vi "Switch Scalar Type.vi"(8 "error in (no error)":errorcluster, 11 "Node Ptr":u64 format="%.0x") -> (0 "error out":errorcluster)   [LabVIEW 2019, in "FPGA Addon System Explorer.lvlib"]
uses:
  FPGA Addon System Explorer.lvlib
  <vilib>/NI VeriStand/Custom Device API/Custom Device Channel.ctl
  <vilib>/NI VeriStand/Custom Device API/Custom Device Channel Type.ctl
  Addon Shared/SubVIs/Constants.vi
  <vilib>/NI VeriStand/Custom Device API/Set Item Property (String).vi
  <vilib>/NI VeriStand/Custom Device API/Get Item Property (String).vi
  <vilib>/NI VeriStand/Custom Device API/Custom Device API.lvlib
  Addon Shared/FPGA Addon Shared.lvlib
  <vilib>/NI VeriStand/Custom Device Tools/Custom Device Utility Library/Custom Device Utility Library.lvlib
  <vilib>/NI VeriStand/Custom Device Tools/Custom Device Utility Library/Search Direction.ctl
  <vilib>/NI VeriStand/Custom Device Tools/Custom Device Utility Library/NI VeriStand - Search for Item by GUID.vi
panel:
  in  "Tag":string
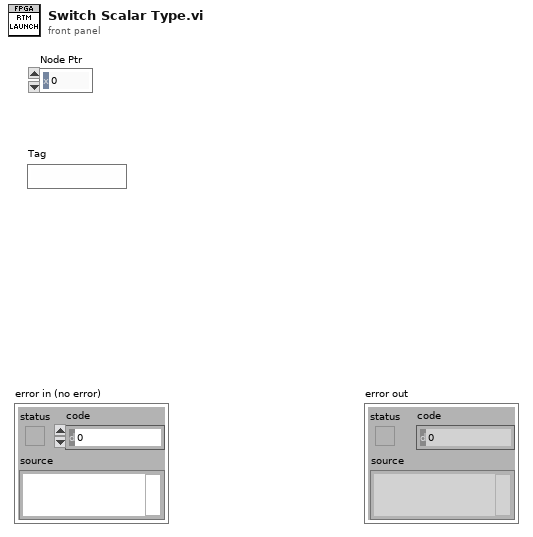
[diagram p1: front panel]
types:
  T1 = typedef "Custom Device Utility Library.lvlib/Search Direction.ctl" = enum16{"Down", "Up"}
  T2 = typedef "Custom Device API.lvlib/Custom Device Item Ref.ctl" = u64
  T3 = typedef "Custom Device API.lvlib/Custom Device Item Info.ctl" = cluster{"Name":string, "Is Channel":bool, "GUID":string, "Is Waveform":bool}
  T4 = typedef "Custom Device API.lvlib/Custom Device Channel.ctl" = cluster{"Type":T5, "Units":string, "Default Value":dbl, "Faultable":bool, "Scalable":bool}
  T5 = typedef "Custom Device API.lvlib/Custom Device Channel Type.ctl" = enum16{"Input", "Output"}
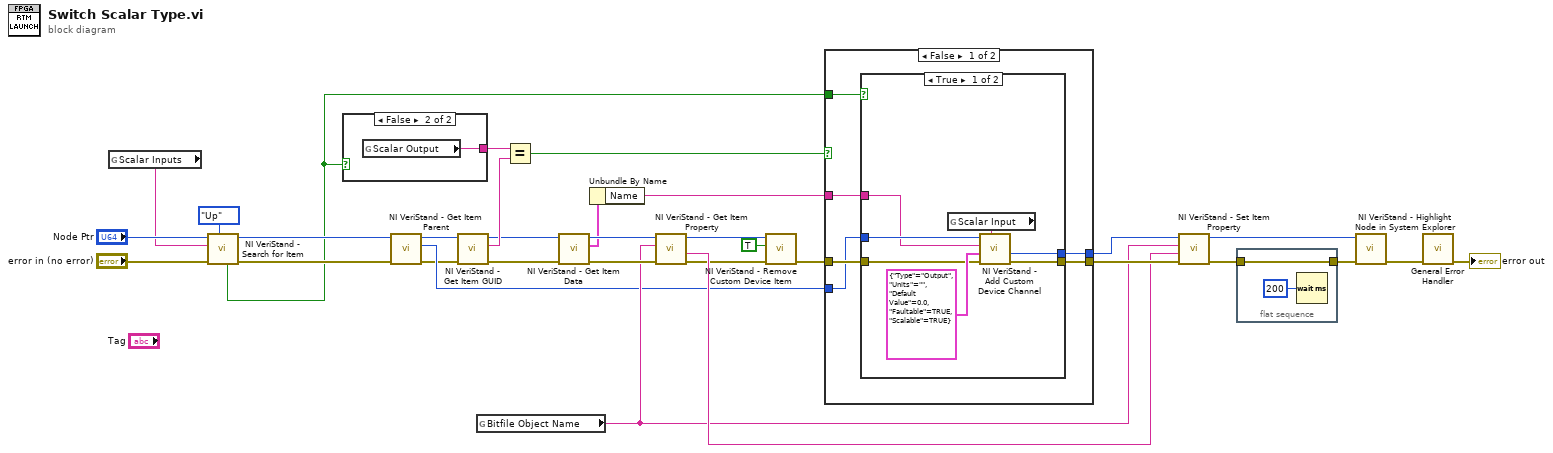
[diagram p0: block diagram]
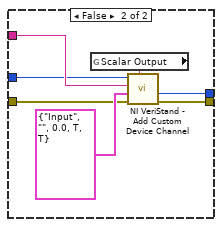
[diagram p2: hidden frame]
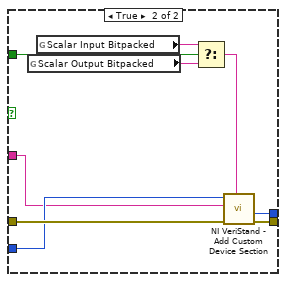
[diagram p3: hidden frame]
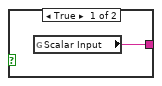
[diagram p4: hidden frame]
diagram:
  n1 = global read "Constants.vi" "Scalar Inputs"() -> (w3:string)
  n2 = call-poly <vilib>:"NI VeriStand - Search for Item.vi"("Direction (Down)"=Search_Direction."Up", "error in"="error in (no error)", "Item GUID"=w3, "Section Ref in"="Node Ptr") -> ("error out"=w5:errorcluster, "Section Ref out"=w4:T2, "Found"=w1:bool)  [unwired: 4 in, 1 out]
  n3 = case shown="False" w1 {
    tunnel: [w33 w34] -> w30
    frame True {
      n4 = global read "Constants.vi" "Scalar Input"() -> (w33:string)
    }
    frame False {
      n5 = global read "Constants.vi" "Scalar Output"() -> (w34:string)
    }
  }
  n6 = call <vilib>:"NI VeriStand - Get Item Parent.vi"("error in (no error)"=w5, "Item Ref in"=w4) -> ("error out"=w8:errorcluster, "Parent Ref"=w9:T2, "Item Ref out"=w29:T2)  [unwired: 6 in, 1 out]
  n7 = call <vilib>:"NI VeriStand - Get Item GUID.vi"("error in (no error)"=w8, "Item Ref in"=w29) -> ("error out"=w18:errorcluster, "GUID"=w32:string, "Item Ref out"=w20:T2)  [unwired: 7 in]
  n8 = global read "Constants.vi" "Bitfile Object Name"() -> (w14:string)
  n9 = Equal?(x=w30, y=w32) -> (x = y?=w26:bool)
  n10 = call <vilib>:"NI VeriStand - Get Item Data.vi"("error in (no error)"=w18, "Item Ref in"=w20) -> ("error out"=w17:errorcluster, "Item Info"=w16:T3, "Item Ref out"=w19:T2)  [unwired: 6 in, 1 out]
  n11 = Unbundle By Name(w16) -> ("Name"=w15:string)
  n12 = call-poly <vilib>:"NI VeriStand - Get Item Property.vi"("error in (no error)"=w17, "Property Name"=w14, "Item Ref in"=w19) -> ("error out"=w22:errorcluster, "Value"=w23:string, "Item Ref out"=w21:T2)  [unwired: 5 in, 1 out]
  n13 = call <vilib>:"NI VeriStand - Remove Custom Device Item.vi"("error in (no error)"=w22, "Force Delete (F)"=TRUE, "Item Ref in"=w21) -> ("error out"=w27:errorcluster)  [unwired: 7 in, 1 out]
  n14 = case shown="False" w26 {
    tunnel: w27 -> [w40 w63]
    tunnel: w9 -> [w36 w62]
    tunnel: w1 -> [w37 w60]
    tunnel: [w39 w58] -> w25
    tunnel: [w38 w57] -> w24
    tunnel: w15 -> [w35 w56]
    frame False {
      n15 = case shown="True" w37 {
        tunnel: w40 -> [w45 w52]
        tunnel: [w44 w51] -> w39
        tunnel: [w43 w50] -> w38
        tunnel: w36 -> [w42 w48]
        tunnel: w35 -> [w41 w49]
        frame True {
          n16 = global read "Constants.vi" "Scalar Input"() -> (w47:string)
          n17 = call <vilib>:"NI VeriStand - Add Custom Device Channel.vi"("GUID (Default Channel)"=w47, "error in (no error)"=w45, "Channel"=T4 {"Type"=enum."Output", "Units"="", "Default Value"=0.0, "Faultable"=TRUE, "Scalable"=TRUE}, "Channel Name"=w41, "Parent Ref in"=w42) -> ("error out"=w44:errorcluster, "Channel Ref"=w43:T2)  [unwired: 3 in, 2 out]
        }
        frame False {
          n18 = global read "Constants.vi" "Scalar Output"() -> (w54:string)
          n19 = call <vilib>:"NI VeriStand - Add Custom Device Channel.vi"("GUID (Default Channel)"=w54, "error in (no error)"=w52, "Channel"=T4 {"Type"=enum."Input", "Units"="", "Default Value"=0.0, "Faultable"=TRUE, "Scalable"=TRUE}, "Channel Name"=w49, "Parent Ref in"=w48) -> ("error out"=w51:errorcluster, "Channel Ref"=w50:T2)  [unwired: 3 in, 2 out]
        }
      }
    }
    frame True {
      n20 = global read "Constants.vi" "Scalar Output Bitpacked"() -> (w59:string)
      n21 = global read "Constants.vi" "Scalar Input Bitpacked"() -> (w61:string)
      n22 = Select(t=w61, s=w60, f=w59) -> (s? t:f=w55:string)
      n23 = call <vilib>:"NI VeriStand - Add Custom Device Section.vi"("GUID (Default Section)"=w55, "error in (no error)"=w63, "Section Name"=w56, "Parent Ref in"=w62) -> ("error out"=w58:errorcluster, "Section Ptr"=w57:T2)  [unwired: 4 in, 2 out]
    }
  }
  n24 = call-poly <vilib>:"NI VeriStand - Set Item Property.vi"("error in (no error)"=w25, "Value"=w23, "Property Name"=w14, "Item Ref in"=w24) -> ("error out"=w10:errorcluster, "Item Ref out"=w12:T2)  [unwired: 5 in, 1 out]
  n25 = flat-sequence {
    tunnel: [w65] -> w11
    tunnel: w10 -> [w65]
    frame #0 {
      n26 = Wait (ms)(milliseconds to wait=u32 200) -> ()  [unwired: 1 out]
    }
  }
  n27 = call <vilib>:"NI VeriStand - Highlight Node in System Explorer.vi"("error in (no error)"=w11, "Item Ref in"=w12) -> ("error out"=w13:errorcluster)  [unwired: 8 in, 1 out]
  n28 = call <vilib>:"General Error Handler.vi"("error in (no error)"=w13) -> ("error out"=→"error out":errorcluster)  [unwired: 10 in, 4 out]
